vi "dT.vi"(8 "error in (no error)":errorcluster, 11 "PID in":refnum<class "PID.lvclass">) -> (0 "error out":errorcluster, 2 "dT":dbl, 3 "PID out":refnum<class "PID.lvclass">)   [LabVIEW 2020, in "IG PID.lvlib" / "PID.lvclass"]
uses:
  PID.lvclass
  PID.lvclass/PID.ctl
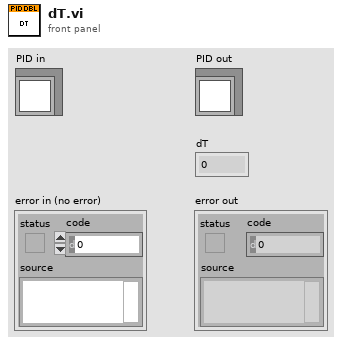
[diagram p1: front panel]
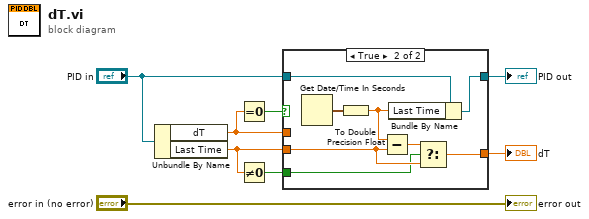
[diagram p0: block diagram]
diagram:
  n1 = Unbundle By Name("PID in") -> ("dT"=w6:dbl, "Last Time"=w2:dbl)
  n2 = Equal To 0?(x=w6) -> (x = 0?=w7:bool)
  n3 = Not Equal To 0?(x=w2) -> (x != 0?=w1:bool)
  n4 = case shown="True" w7 {
    tunnel: w6 -> [w10 _]
    tunnel: w2 -> [_ w13]
    tunnel: [w10 w11] -> w5
    tunnel: "PID in" -> [w9 w17]
    tunnel: [w9 w15] -> w3
    tunnel: w1 -> [_ w12]
    frame False {
    }
    frame True {
      n5 = Get Date/Time In Seconds() -> (seconds since 1Jan1904=w18:timestamp)
      n6 = To Double Precision Float(number=w18) -> (double precision float=w16:dbl)
      n7 = Subtract(x=w16, y=w13) -> (x-y=w14:dbl)
      n8 = Bundle By Name(cluster=w17, "Last Time"=w16) -> (w15:refnum<class "PID.lvclass">)
      n9 = Select(t=w14, s=w12, f=w13) -> (s? t:f=w11:dbl)
    }
  }
  "PID out" <- w3
  "dT" <- w5
  "error out" <- "error in (no error)"
